vi "RDC-water-generate_perm_from_freq.vi"(10 "Frequency":dbl[](array[numeric]), 11 "water Temp (25C) [10-40C]":dbl=25.0) -> (0 "used temp":dbl, 1 "Complex Perm":cluster{dbl[], cdb[]}, 2 "Imag Perm":cluster{dbl[], dbl[]}, 3 "Real Perm":cluster{dbl[], dbl[]}, 4 "Complex perm":cdb[](array[numeric]))   [LabVIEW 2020, in "RDC-Reflection_Data_Computation.lvlib"]
doc: "Generates the water model permittivity for the given frequency array at the given water temperature (10-40 C), using RDC-water-generate_perm."
uses:
  RDC-Reflection_Data_Computation.lvlib
panel:
  out "size(s) 2":i32
  out "size(s)":i32
  out "loss":cluster{dbl[], dbl[]}(graph)
  out "perm":cluster{dbl[], dbl[]}(graph)
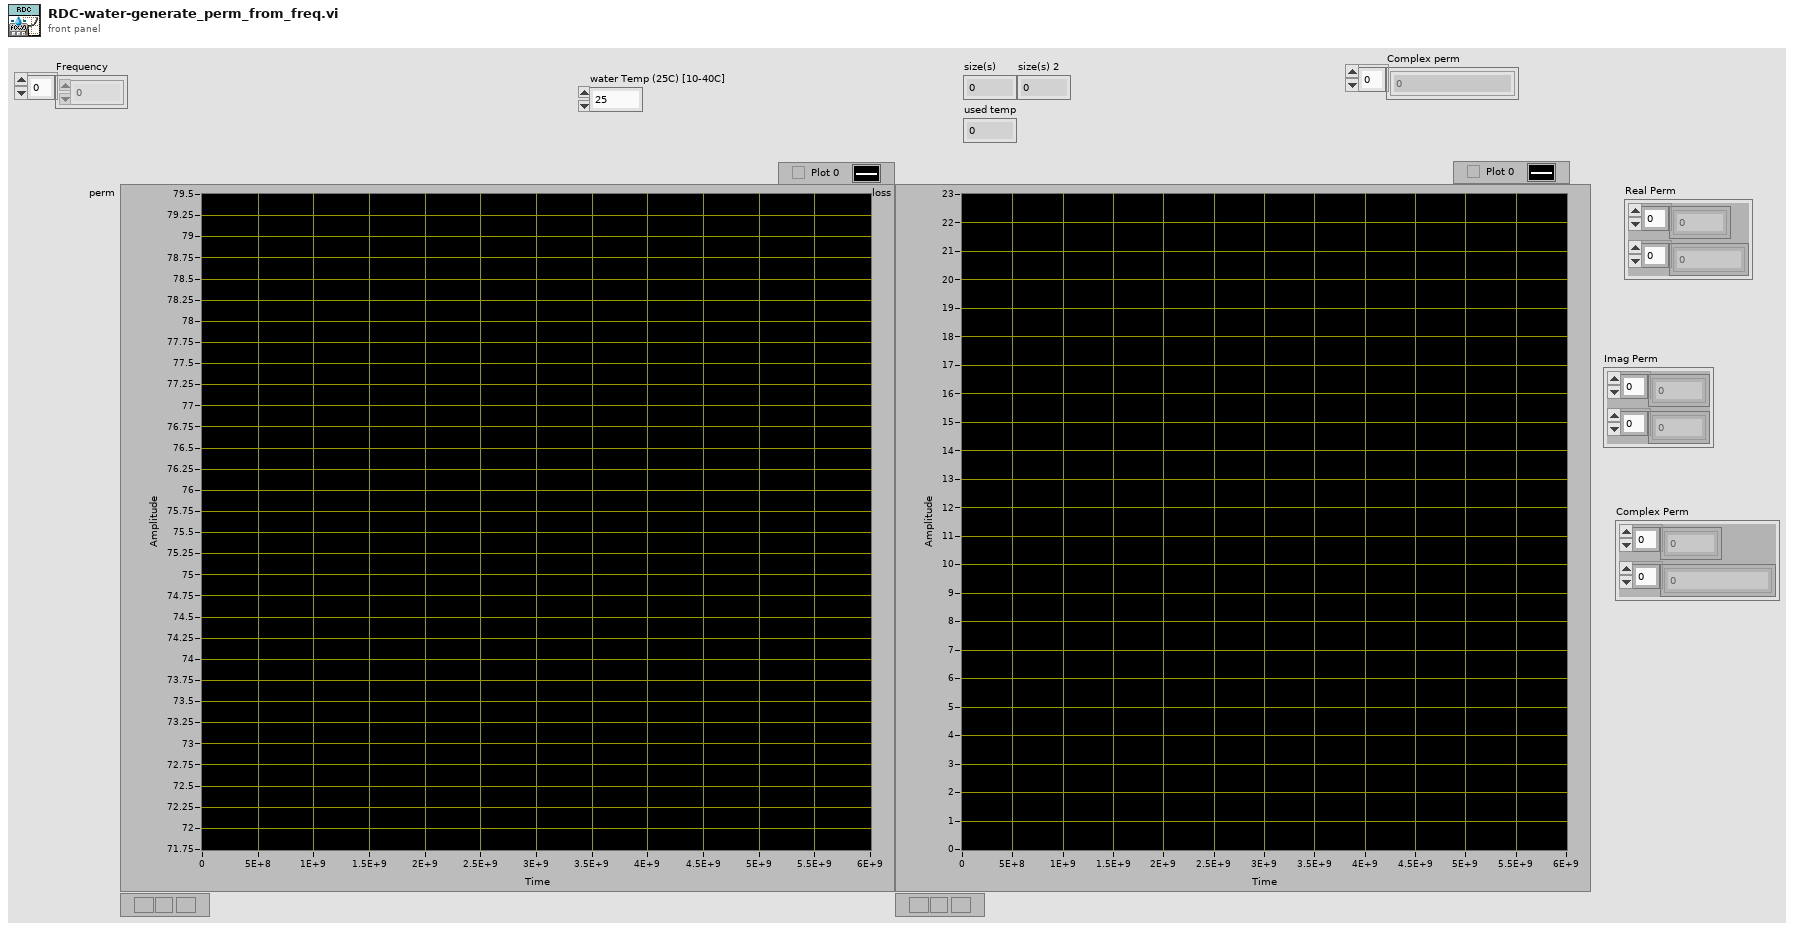
[diagram p1: front panel]
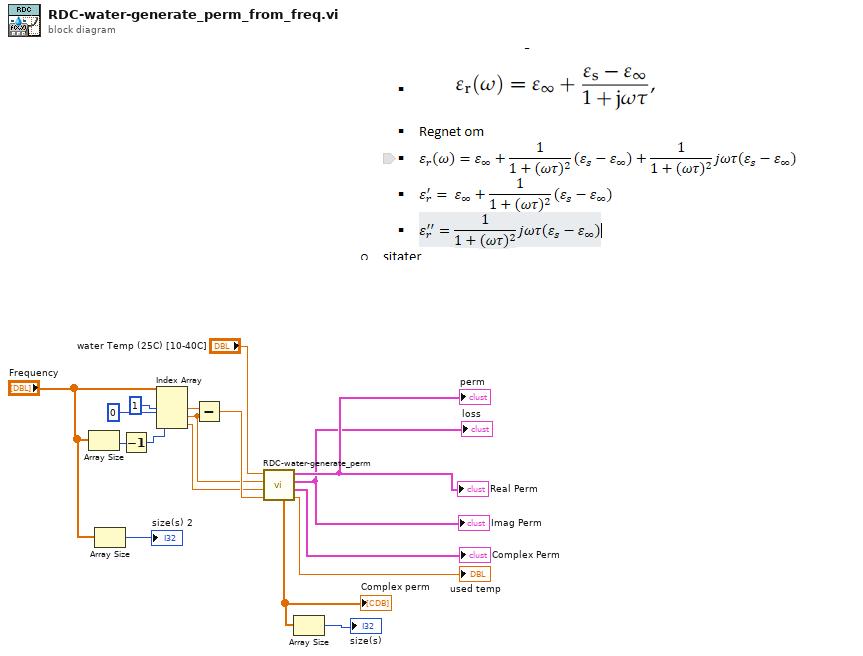
[diagram p0: block diagram]
diagram:
  n1 = Array Size(array="Frequency") -> (size(s)=w15:i32)
  n2 = Array Size(array="Frequency") -> (size(s)=→"size(s) 2":i32)
  n3 = Decrement(x=w15) -> (x-1=w14:i32)
  n4 = Index Array(array="Frequency", index #1=1 ("index"), index #2=0 ("index"), index #3=w14) -> (element #1=w13:dbl, element #2=w10:dbl, element #3=w9:dbl)
  n5 = Subtract(x=w13, y=w10) -> (x-y=w11:dbl)
  n6 = call "RDC-water-generate_perm.vi"("Increment f (10MHz)"=w11, "Stop f (6GHz) 2"=w9, "Start f (300MHz)"=w10, "water Temp (25C) [10-40C]"="water Temp (25C) [10-40C]") -> ("used temp"=→"used temp":dbl, "Complex Perm"=→"Complex Perm":cluster{dbl[], cdb[]}, "Imag Perm"=→"Imag Perm" →"loss":cluster{dbl[], dbl[]}, "Real Perm"=→"Real Perm" →"perm":cluster{dbl[], dbl[]}, "Complex perm"=w5:cdb[])  [unwired: 3 in]
  "Complex perm" <- w5
  n7 = Array Size(array=w5) -> (size(s)=→"size(s)":i32)
